vi "PicoScope5000aSetRapidSegments.vi"(5 "RapidBlock":bool=TRUE, 7 "nSegments":T1 format="%.4p", 8 "error in (no error)":errorcluster, 11 "handle in":i16) -> (0 "error out":errorcluster, 3 "handle out":i16, 6 "nCaptures":u64)   [LabVIEW 2010]
doc: "Calls ps5000aMemorySegments, and ps5000aSetNoOfCaptures"
uses:
  ps5000a.dll
  shared/nSegments.ctl
panel:
  out "nMaxSamples":u64
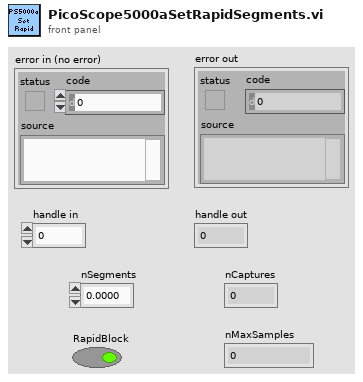
[diagram p1: front panel]
types:
  T1 = typedef "nSegments.ctl" = u64
  T2 = cluster{"status":bool, "code":u32, "source":string}
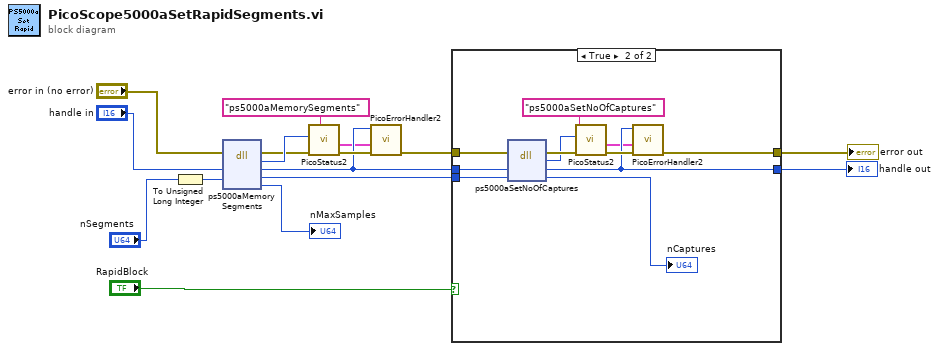
[diagram p0: block diagram]
diagram:
  n1 = To Unsigned Long Integer(number="nSegments") -> (unsigned 32bit integer=w3:u32)
  n2 = dll-call lib="ps5000a.dll" fn="ps5000aMemorySegments" ("ps3000.dll:_ps3000_open_unit@0")(error in="error in (no error)", "handle"="handle in", "nSegments"=w3) -> (error out=w15:errorcluster, "PICO_STATUS"=w16:u32, "handle"=w11:i16, "nSegments"=w13:u32, "nMaxSamples"=→"nMaxSamples":i32)  [unwired: 3 in, 1 out]
  n3 = call "PicoStatus2.vi"("PICO source"="ps5000aMemorySegments" ("source"), "Error in"=w15, "PICO STATUS"=w16) -> ("error out"=w12:errorcluster, "PICO_STATUS out"=w1:T2)  [unwired: 5 in]
  n4 = call "PicoErrorHandler2.vi"("error in (no error)"=w12, "PICO_STATUS in"=w1, "handle In"=w11) -> ("error out"=w9:errorcluster)  [unwired: 8 in]
  n5 = case shown="True" "RapidBlock" {
    tunnel: w13 -> [_ w29]
    tunnel: w11 -> [w17 w26]
    tunnel: w9 -> [w18 w23]
    tunnel: [w18 w22] -> w6
    tunnel: [w17 w21] -> w5
    frame False {
    }
    frame True {
      n6 = dll-call lib="ps5000a.dll" fn="ps5000aSetNoOfCaptures" ("ps3000.dll:_ps3000_open_unit@0")(error in=w23, "handle"=w26, "nCaptures"=w29) -> (error out=w28:errorcluster, "PICO_STATUS"=w24:u32, "handle"=w21:i16, "nCaptures"=→"nCaptures":u32)  [unwired: 2 in, 1 out]
      n7 = call "PicoStatus2.vi"("PICO source"="ps5000aSetNoOfCaptures" ("source"), "Error in"=w28, "PICO STATUS"=w24) -> ("error out"=w25:errorcluster, "PICO_STATUS out"=w19:T2)  [unwired: 5 in]
      n8 = call "PicoErrorHandler2.vi"("error in (no error)"=w25, "PICO_STATUS in"=w19, "handle In"=w21) -> ("error out"=w22:errorcluster)  [unwired: 8 in]
    }
  }
  "error out" <- w6
  "handle out" <- w5
